vi "Update CAN Status.vi"(8 "error in (no error)":errorcluster, 11 "CAN_Reader_NIXNET_Plugin":refnum<class "CAN_Reader_NIXNET_Plugin.lvclass">) -> (0 "error out":errorcluster, 3 "CAN_Reader_NIXNET_Plugin":refnum<class "CAN_Reader_NIXNET_Plugin.lvclass">)   [LabVIEW 2021, in "CAN_Reader_NIXNET_Plugin.lvclass"]
uses:
  CAN_Reader_NIXNET_Plugin.lvclass
  CAN_Reader_NIXNET_Plugin.lvclass/CAN_Reader_NIXNET_Plugin.ctl
  <vilib>/CIF Foundation/CIF XNET CAN RW/XNET CAN RW.lvclass
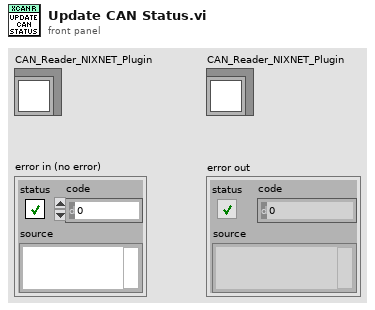
[diagram p1: front panel]
types:
  T1 = typedef "CAN_RW_CORE.lvclass/CAN Status.ctl" = cluster{"Comm State":T2, "Last Error":T3, "RX Error Counter":u8, "TX Error Counter":u8}
  T2 = typedef "CAN_RW_CORE.lvclass/Communication State.ctl" = enum16{"Error Active", "Error Passive", "Bus Off"}
  T3 = typedef "CAN_RW_CORE.lvclass/Last Error.ctl" = enum16{"None", "Stuff", "Form", "Ack", "Bit1", "Bit0", "CRC", "Unknown"}
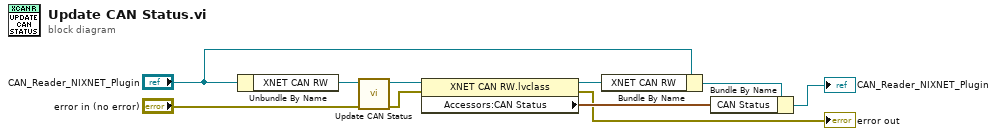
[diagram p0: block diagram]
diagram:
  n1 = Unbundle By Name("CAN_Reader_NIXNET_Plugin") -> ("XNET CAN RW"=w9:refnum<class "XNET CAN RW.lvclass">)
  n2 = call <vilib>:"Update CAN Status.vi"("error in (no error)"="error in (no error)", "XNET CAN RW in"=w9) -> ("error out"=w7:errorcluster, "XNET CAN RW out"=w8:refnum<class "XNET CAN RW.lvclass">)  [unwired: 8 in]
  n3 = property class="XNET CAN RW.lvclass"(reference=w8, error in=w7) -> (reference out=w6:refnum<class "XNET CAN RW.lvclass">, error out=→"error out":errorcluster, "Accessors:CAN Status"=w4:T1)
  n4 = Bundle By Name(cluster="CAN_Reader_NIXNET_Plugin", "XNET CAN RW"=w6) -> (w5:refnum<class "CAN_Reader_NIXNET_Plugin.lvclass">)
  n5 = Bundle By Name(cluster=w5, "CAN Status"=w4) -> (→"CAN_Reader_NIXNET_Plugin":refnum<class "CAN_Reader_NIXNET_Plugin.lvclass">)
